vi "Close.vi"(8 "error in (no error)":errorcluster, 11 "DBC in":refnum<class "DBC.lvclass">) -> (0 "error out":errorcluster)   [LabVIEW 2020, in "ORM_sqlite_jdp.lvlib" / "DBC.lvclass"]
uses:
  DBC.lvclass
  DBC.lvclass/DBC.ctl
  <vilib>/Viviota/shared/ORM.lvlibp/DbConnection/DbConnection.lvclass
  <vilib>/drjdpowell/SQLite Library/SQL Connection/Connection.lvclass
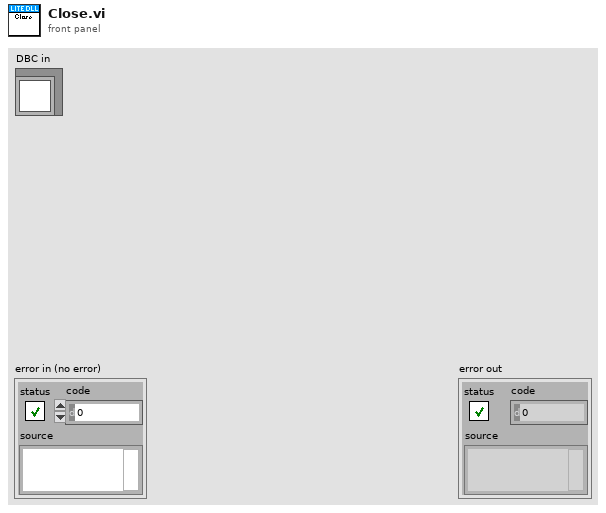
[diagram p1: front panel]
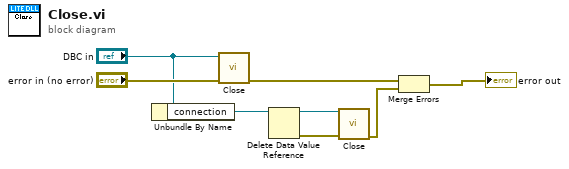
[diagram p0: block diagram]
diagram:
  n1 = Unbundle By Name("DBC in") -> ("connection"=w3:refnum<data-value>)
  n2 = call-parent "Close.vi"("error in (no error)"="error in (no error)", "DbConnection in"="DBC in") -> ("error out"=w8:errorcluster)  [unwired: 9 in]
  n3 = Delete Data Value Reference(data value reference=w3) -> (data value=w2:refnum<class "Connection.lvclass">, error out=w1:errorcluster)  [unwired: 1 in]
  n4 = call-dynamic "Close.vi"("error in (no error)"=w1, "SQLite Connection in"=w2) -> ("error out"=w4:errorcluster)  [unwired: 9 in]
  n5 = Merge Errors(w8, w4) -> (→"error out":errorcluster)
